vi "Convert JSON to Unicode text.vi"(4 "String in":string, 5 "Unicode (True)":bool=TRUE) -> (1 "String out":string)   [LabVIEW 2019, in "Language Selection.lvlib"]
doc: "- - -\nCopyright (c) 2026, Merecs Engineering GmbH"
uses:
  Language Selection.lvlib
  <vilib>/addons/Tools/Unicode/_subVIs/Convert ASCII to UTF-16LE (Scalar).vi
  <vilib>/addons/Tools/Unicode/UI Unicode Tools.lvlib
panel:
  # "Connector Pane"
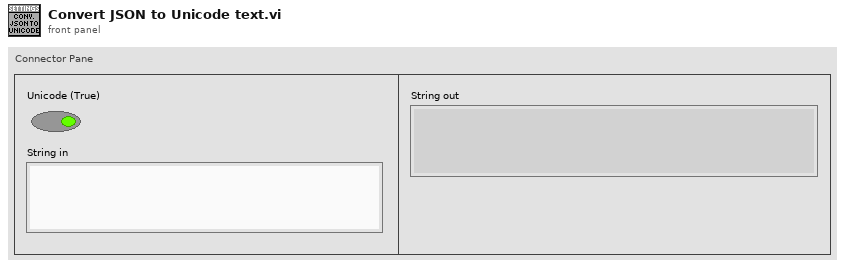
[diagram p1: front panel]
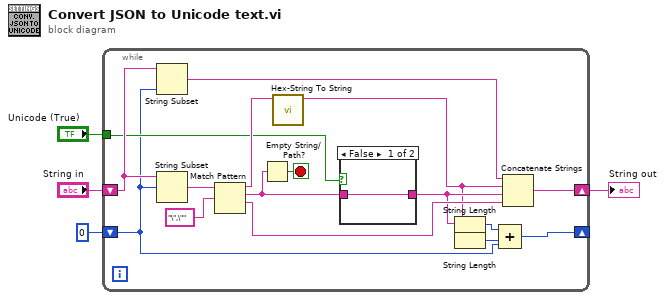
[diagram p0: block diagram]
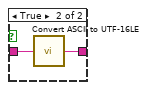
[diagram p2: hidden frame]
diagram:
  n1 = while {
    shift-right: [w18] -> w2
    shift-left: "String in" -> [w10]
    shift-right: [w12] -> _
    shift-left: 0 ("offset past match") -> [w5]
    tunnel: "Unicode (True)" -> [w7]
    stop <- w16 stop-if-true
    n2 = String Subset(string=w10, length (rest)=w5) -> (substring=w11:string)  [unwired: 1 in]
    n3 = String Subset(string=w10, offset (0)=w5) -> (substring=w9:string)  [unwired: 1 in]
    n4 = Match Pattern(string=w9, regular expression="\",\"") -> (before substring=w8:string, match substring=w17:string, after substring=w19:string)  [unwired: 1 in, 1 out]
    n5 = Empty String/Path?(string/path=w17) -> (empty?=w16:bool)
    n6 = call "Hex-String To String.vi"("HEX-String"=w8) -> ("string"=w6:string)  [unwired: 10 in]
    n7 = case shown="False" w7 {
      tunnel: w17 -> [w21 w23]
      tunnel: [w21 w22] -> w15
      frame False {
      }
      frame True {
        n8 = call-poly <vilib>:"Convert ASCII to UTF-16LE.vi"("ASCII"=w23) -> ("Unicode"=w22:string)  [unwired: 4 in]
      }
    }
    n9 = String Length(string=w15) -> (length=w13:i32)
    n10 = String Length(string=w6) -> (length=w14:i32)
    n11 = Compound Arithmetic op=ADD(w13, w14, w5) -> (w12:i32)
    n12 = Concatenate Strings(w11, w6, w15, w19) -> (w18:string)
  }
  "String out" <- w2
